vi "binairo.vi"() -> ()   [LabVIEW 2026]
uses:
  <vilib>/picture/picture.llb/imagedata.ctl
panel:
  out "error":bool
  in  "thr 0":i32=90
  in  "thr empty":i32=88
  in  "thr 1":i32=90
  out "command":string
  out "grid string":string
  out "grid error":bool
  out "# cols":i32
  out "#rows":i32
  in  "error in":errorcluster
  out "error out":errorcluster
  out "Cell values":string
  out "standard error":string
  out "standard output":string
  out "1-bit cell image":bool[][](array[boolean])
  out "cell":picture
  out "B&W picture":picture
  out "image data":T1
  out "1-bit pixmap":bool[][](array[boolean])
  out "color Picture":picture
  in  "PNG Path":path
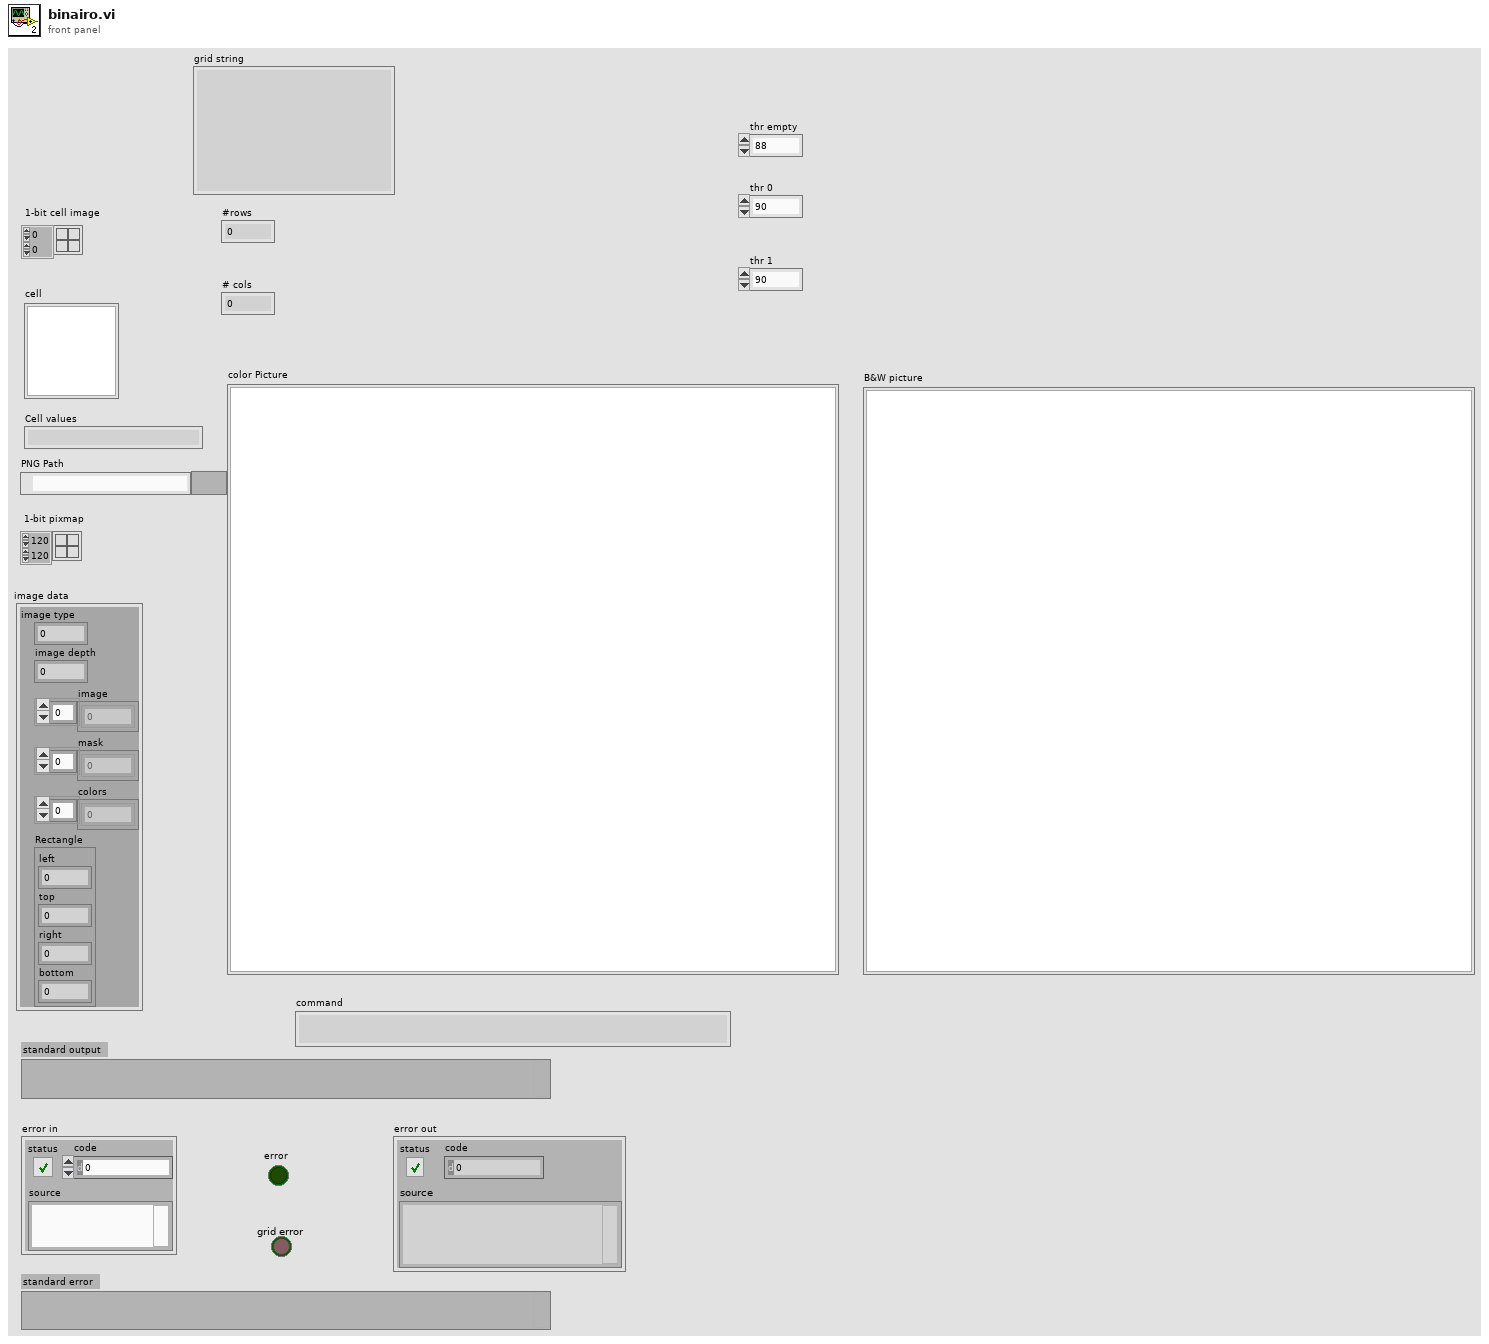
[diagram p1: front panel]
types:
  T1 = typedef "imagedata.ctl" = cluster{"image type":i32, "image depth":i32, "image":u8[], "mask":u8[], "colors":u32[], "Rectangle":cluster{"left":i16, "top":i16, "right":i16, "bottom":i16}}
  T2 = enum16{"big-endian, network order", "native, host order", "little-endian"}
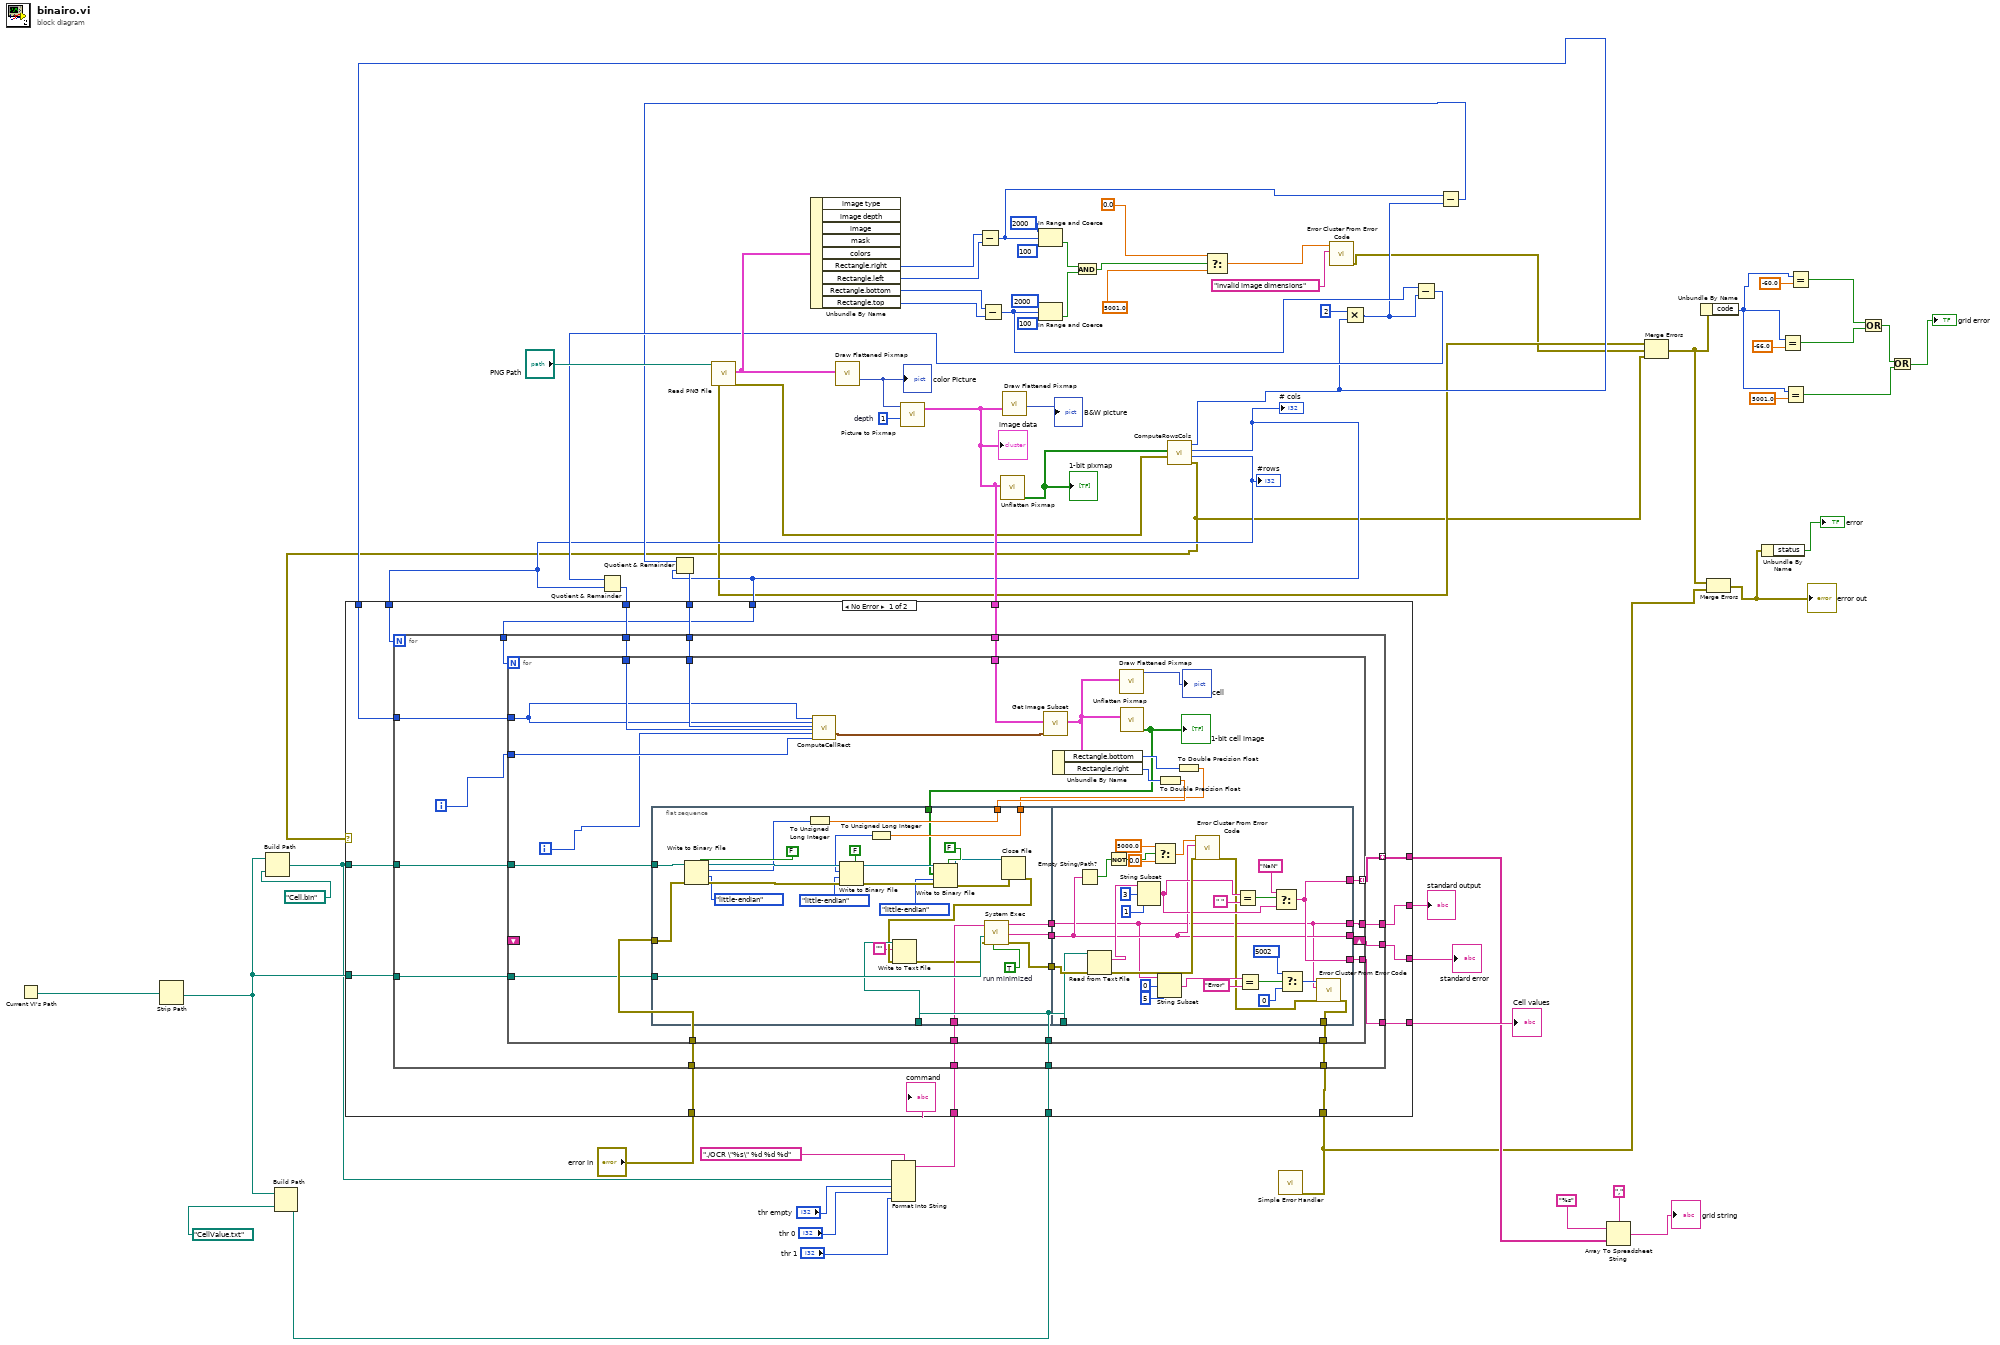
[diagram p0: block diagram]
diagram:
  w66 = 1  # depth
  n1 = Current VI's Path() -> (path=w44:path)
  n2 = Strip Path(path=w44) -> (stripped path=w41:path)  [unwired: 1 out]
  n3 = Build Path(base path=w41, name or relative path=path "Cell.bin") -> (appended path=w38:path)
  n4 = Build Path(base path=w41, name or relative path=path "CellValue.txt") -> (appended path=w47:path)
  n5 = call <vilib>:"Read PNG File.vi"("path to PNG file"="PNG Path") -> ("error out"=w17:errorcluster, "image data"=w64:T1)  [unwired: 8 in, 1 out]
  n6 = Unbundle By Name(w64) -> ("Rectangle.right"=w36:i16, "Rectangle.left"=w51:i16, "Rectangle.bottom"=w1:i16, "Rectangle.top"=w52:i16)  [unwired: 5 out]
  n7 = call <vilib>:"Draw Flattened Pixmap.vi"("image data"=w64) -> ("new picture"=w67:picture)  [unwired: 8 in]
  "color Picture" <- w67
  n8 = Format Into String "Format Into String"(format string="./OCR \"%s\" %d %d %d" ("initial string"), w38, "thr empty", "thr 0", "thr 1") -> (resulting string=w39:string)  [unwired: 2 in, 1 out]
  n9 = call <vilib>:"Picture to Pixmap.vi"("depth"=w66, "picture"=w67) -> ("image data"=w37:T1)  [unwired: 8 in, 1 out]
  "image data" <- w37
  n10 = Subtract(x=w36, y=w51) -> (x-y=w28:i16)
  n11 = Subtract(x=w1, y=w52) -> (x-y=w31:i16)
  n12 = call <vilib>:"Unflatten Pixmap.vi"("image data"=w37) -> ("1-bit pixmap"=w2:bool[][])  [unwired: 4 in, 6 out]
  "1-bit pixmap" <- w2
  n13 = call <vilib>:"Draw Flattened Pixmap.vi"("image data"=w37) -> ("new picture"=→"B&W picture":picture)  [unwired: 8 in]
  n14 = In Range and Coerce(upper limit=i16 2000, x=w28, lower limit=i16 100) -> (In Range?=w59:bool)  [unwired: 1 out]
  n15 = In Range and Coerce(upper limit=i16 2000, x=w31, lower limit=i16 100) -> (In Range?=w58:bool)  [unwired: 1 out]
  n16 = And(x=w59, y=w58) -> (x .and. y?=w56:bool)
  n17 = call "ComputeRowsCols.vi"("error in (no error)"=w17, "1-bit pixmap"=w2) -> ("error out"=w3:errorcluster, "#rows"=w19:i32, "# cols"=w18:i32, "origin"=w25:i32)  [unwired: 6 in]
  "#rows" <- w19
  "# cols" <- w18
  n18 = Select(t=0.0, s=w56, f=5001.0) -> (s? t:f=w54:dbl)
  n19 = call <vilib>:"Error Cluster From Error Code.vi"("error message (\"\")"="invalid image dimensions", "error code (0)"=w54) -> ("error out"=w16:errorcluster)  [unwired: 7 in]
  n20 = Multiply(x=2, y=w25) -> (x*y=w27:i32)
  n21 = Subtract(x=w31, y=w27) -> (x-y=w29:i32)
  n22 = Quotient & Remainder(x=w29, y=w19) -> (floor(x/y)=w30:i32)  [unwired: 1 out]
  n23 = Subtract(x=w28, y=w27) -> (x-y=w26:i32)
  n24 = Quotient & Remainder(x=w26, y=w18) -> (floor(x/y)=w35:i32)  [unwired: 1 out]
  n25 = case shown="No Error" w3 {
    tunnel: "error in" -> [w84 _]
    tunnel: [w83 _] -> w49
    tunnel: [w82 _] -> w48
    tunnel: w47 -> [w81 _]
    tunnel: [w80 _] -> w4
    tunnel: [w79 _] -> w42
    tunnel: w41 -> [w78 _]
    tunnel: w39 -> [w77 _]
    tunnel: w38 -> [w76 _]
    tunnel: w37 -> [w75 _]
    tunnel: w35 -> [w74 _]
    tunnel: [w73 _] -> w34
    tunnel: w30 -> [w72 _]
    tunnel: w25 -> [w71 _]
    tunnel: w19 -> [w70 _]
    tunnel: w18 -> [w69 _]
    frame No Error {
      n26 = for {
        N: w70 -> [_]
        tunnel: w84 -> [w100]
        tunnel: [w97] -> w83
        tunnel: [w99] -> w82
        tunnel: w81 -> [w98]
        tunnel: [w96] -> w80
        tunnel: [w95] -> w79
        tunnel: w78 -> [w94]
        tunnel: w76 -> [w93]
        tunnel: w77 -> [w92]
        tunnel: w75 -> [w91]
        tunnel: w72 -> [w90]
        tunnel: w74 -> [w89]
        tunnel: [w88] -> w73 mode=indexing
        tunnel: w71 -> [w87]
        tunnel: w69 -> [w86]
        i -> [w85]
        n27 = for {
          N: w86 -> [_]
          tunnel: [w126] -> w99
          shift-right: [w127] -> w97
          shift-left: _ -> [_]
          tunnel: w98 -> [w102]
          tunnel: w100 -> [w121]
          tunnel: [w122] -> w96
          tunnel: [w120] -> w95
          tunnel: w94 -> [w119]
          tunnel: w93 -> [w116]
          tunnel: w92 -> [w115]
          tunnel: w91 -> [w114]
          tunnel: w90 -> [w105]
          tunnel: w89 -> [w106]
          tunnel: [w108] -> w88 mode=indexing
          tunnel: w87 -> [w103]
          tunnel: w85 -> [w104]
          i -> [w101]
          n28 = flat-sequence {
            tunnel: [w156] -> w125
            tunnel: [w155] -> w124
            tunnel: [w154] -> w123
            tunnel: w121 -> [w151]
            tunnel: w110 -> [w153]
            tunnel: w109 -> [w152]
            tunnel: w112 -> [w146]
            tunnel: w119 -> [w145]
            tunnel: w116 -> [w144]
            tunnel: w115 -> [w143]
            tunnel: w102 -> [w130]
            tunnel: [w157] -> w126
            tunnel: [w158] -> w127
            tunnel: w125 -> [w158]
            tunnel: w124 -> [w157]
            tunnel: w123 -> [w184]
            tunnel: w102 -> [w180]
            tunnel: [w159] -> w122
            tunnel: [w169] -> w120
            tunnel: [w169] -> w108
            frame #0 {
              w134 = TRUE  # run minimized
              n29 = To Unsigned Long Integer(number=w153) -> (unsigned 32bit integer=w133:u32)
              n30 = Write to Binary File(file (use dialog)=w144, data=w133, error in=w151, 5:FALSE ("prepend array or string size? (T)"), 9:T2."little-endian" ("byte order (0:big-endian, network order)")) -> (refnum out=w148:refnum<file>, error out=w150:errorcluster)  [unwired: 1 in, 1 out]
              n31 = To Unsigned Long Integer(number=w152) -> (unsigned 32bit integer=w132:u32)
              n32 = Write to Binary File(file (use dialog)=w148, data=w132, error in=w150, 5:FALSE ("prepend array or string size? (T)"), 9:T2."little-endian" ("byte order (0:big-endian, network order)")) -> (refnum out=w147:refnum<file>, error out=w149:errorcluster)  [unwired: 1 in, 1 out]
              n33 = Write to Binary File(file (use dialog)=w147, data=w146, error in=w149, 5:FALSE ("prepend array or string size? (T)"), 9:T2."little-endian" ("byte order (0:big-endian, network order)")) -> (refnum out=w139:refnum<file>, error out=w138:errorcluster)  [unwired: 1 in, 1 out]
              n34 = Close File(refnum=w139, error in=w138) -> (error out=w129:errorcluster)  [unwired: 1 out]
              n35 = Write to Text File(file (use dialog)=w130, text="", error in=w129) -> (error out=w131:errorcluster)  [unwired: 1 in, 2 out]
              n36 = call <vilib>:"System Exec.vi"("run minimized? (F)"=w134, "error in (no error)"=w131, "working directory"=w145, "command line"=w143) -> ("error out"=w154:errorcluster, "standard error"=w156:string, "standard output"=w155:string)  [unwired: 4 in, 1 out]
            }
            frame #1 {
              n37 = Empty String/Path?(string/path=w158) -> (empty?=w179:bool)
              n38 = Read from Text File(file (use dialog)=w180, error in=w184) -> (text=w181:string, error out=w174:errorcluster)  [unwired: 2 in, 2 out]
              n39 = Not(x=w179) -> (.not. x?=w178:bool)
              n40 = String Subset(string=w181, offset (0)=3, length (rest)=1 ("length (rest)")) -> (substring=w170:string)
              n41 = Select(t=5000.0, s=w178, f=0.0) -> (s? t:f=w175:dbl)
              n42 = String Subset(string=w157, offset (0)=0, length (rest)=5 ("length (rest)")) -> (substring=w166:string)
              n43 = call <vilib>:"Error Cluster From Error Code.vi"("error in (no error)"=w174, "error message (\"\")"=w158, "error code (0)"=w175) -> ("error out"=w160:errorcluster)  [unwired: 6 in]
              n44 = Equal?(x=w170, y=" ") -> (x = y?=w172:bool)
              n45 = Equal?(x=w166, y="Error") -> (x = y?=w164:bool)
              n46 = Select(t="NaN", s=w172, f=w170) -> (s? t:f=w169:string)
              n47 = Select(t=5002, s=w164, f=0) -> (s? t:f=w161:i32)
              n48 = call <vilib>:"Error Cluster From Error Code.vi"("error in (no error)"=w160, "error message (\"\")"=w157, "error code (0)"=w161) -> ("error out"=w159:errorcluster)  [unwired: 6 in]
            }
          }
          n49 = call "ComputeCellRect.vi"("border X"=w103, "Border Y"=w103, "cell width"=w106, "cell height"=w105, "col idx"=w101, "line idx"=w104) -> ("subset rect"=w107:cluster{i32, i32, i32, i32})  [unwired: 13 in]
          n50 = call <vilib>:"Get Image Subset.vi"("subset rect"=w107, "image data"=w114) -> ("image subset"=w111:T1)  [unwired: 4 in, 1 out]
          n51 = Unbundle By Name "Unbundle By Name"(w111) -> ("Rectangle.bottom"=w118:i16, "Rectangle.right"=w117:i16)
          n52 = call <vilib>:"Draw Flattened Pixmap.vi"("image data"=w111) -> ("new picture"=→"cell":picture)  [unwired: 8 in]
          n53 = call <vilib>:"Unflatten Pixmap.vi"("image data"=w111) -> ("1-bit pixmap"=w112:bool[][])  [unwired: 4 in, 6 out]
          "1-bit cell image" <- w112
          n54 = To Double Precision Float(number=w117) -> (double precision float=w110:dbl)
          n55 = To Double Precision Float(number=w118) -> (double precision float=w109:dbl)
        }
      }
      "command" <- w77
    }
    frame Error {
    }
  }
  "standard output" <- w48
  "standard error" <- w49
  "Cell values" <- w42
  n56 = call <vilib>:"Simple Error Handler.vi"("error in (no error)"=w4) -> ()  [unwired: 4 in, 5 out]
  n57 = Array To Spreadsheet String(delimiter (Tab)=",", array=w34, 3:"%s" ("format string")) -> (spreadsheet string=→"grid string":string)
  n58 = Merge Errors ("Merge Errors for")(w17, w16, w3) -> (w6:errorcluster)
  n59 = Unbundle By Name(w6) -> ("code"=w12:i32)
  n60 = Merge Errors(w6, w4) -> (w5:errorcluster)
  "error out" <- w5
  n61 = Unbundle By Name(w5) -> ("status"=→"error":bool)
  n62 = Equal?(x=w12, y=-66.0) -> (x = y?=w10:bool)
  n63 = Equal?(x=w12, y=5001.0) -> (x = y?=w9:bool)
  n64 = Equal?(x=w12, y=-60.0) -> (x = y?=w11:bool)
  n65 = Or(x=w11, y=w10) -> (x .or. y?=w8:bool)
  n66 = Or(x=w8, y=w9) -> (x .or. y?=→"grid error":bool)
